vi "Read_database.vi"(7 "condition":string, 8 "error in (no error)":errorcluster caption="错误输入（无错误）", 9 "columns":string[](array[string]), 10 "table":string, 11 "Database_access 输入":refnum<class "Database_access.lvclass">) -> (0 "error out":errorcluster caption="错误输出", 2 "data":variant[][](array[variant]), 3 "Database_access 输出":refnum<class "Database_access.lvclass">)   [LabVIEW 2025, in "Database_access.lvclass"]
uses:
  Database_access.lvclass
  Database_access.lvclass/Database_access.ctl
  <vilib>/addons/database/NI_Database_API.lvlib
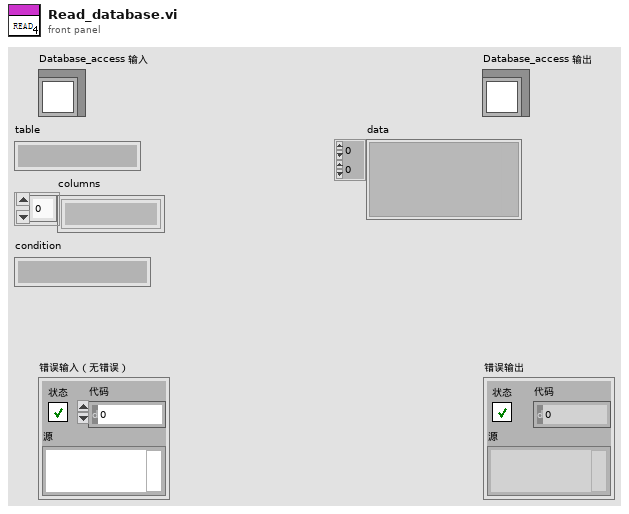
[diagram p1: front panel]
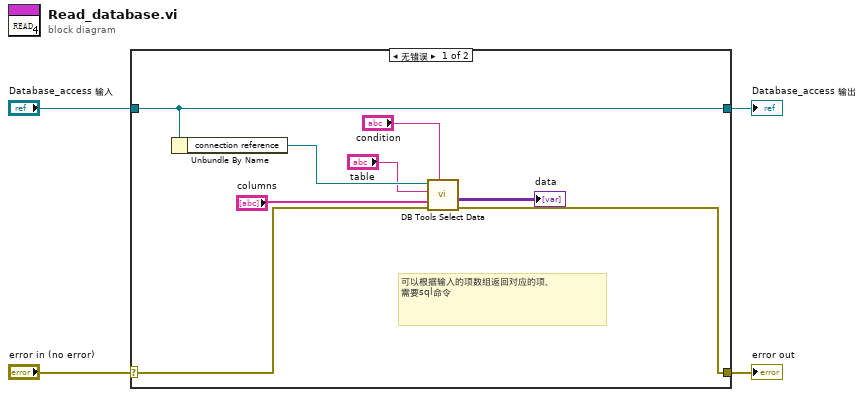
[diagram p0: block diagram]
diagram:
  n1 = case shown="无错误" "error in (no error)" {
    selector: "error in (no error)" -> [w8 w14]
    tunnel: [w7 w14] -> w3
    tunnel: [w12 w13] -> w1
    tunnel: "Database_access 输入" -> [w12 w13]
    frame No Error {
      # "可以根据输入的项数组返回对应的项、\n需要sql命令"
      n2 = Unbundle By Name(w12) -> ("connection reference"=w11:refnum<k1>)
      n3 = call <vilib>:"DB Tools Select Data.vi"("condition"="condition", "error in (no error)"=w8, "columns"="columns", "table"="table", "connection reference"=w11) -> ("error out"=w7:errorcluster, "data"=→"data":variant[][])  [unwired: 1 in, 1 out]
    }
    frame Error {
    }
  }
  "error out" <- w3
  "Database_access 输出" <- w1
